vi "libssh2_agent_free.vi"(8 "error in (no error)":errorcluster, 11 "agent":T1) -> (0 "error out":errorcluster)   [LabVIEW 2017, in "libssh2.lvlib"]
doc: "Release memory associated with an SSH agent handle."
uses:
  libssh2.lvlib
  Agent Refnum.ctl
  Global Settings.vi
  Read Session Refnum.vi
  <vilib>/Utility/semaphor.llb/Acquire Semaphore.vi
  <vilib>/Utility/semaphor.llb/Release Semaphore.vi
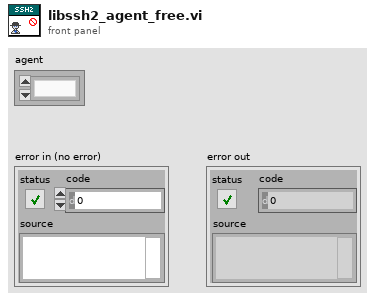
[diagram p1: front panel]
types:
  T1 = typedef "libssh2.lvlib/Agent Refnum.ctl" = refnum<k1>
  T2 = typedef "libssh2.lvlib/Session Refnum.ctl" = refnum<k1>
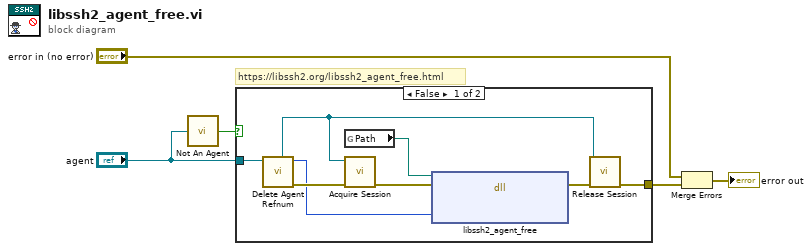
[diagram p0: block diagram]
diagram:
  # "https://libssh2.org/libssh2_agent_free.html"
  n1 = call "Not An Agent.vi"("agent"="agent") -> ("Not a Agent?"=w3:bool)
  n2 = case shown="False" w3 {
    tunnel: [w7 _] -> w5
    tunnel: "agent" -> [w9 _]
    frame False {
      n3 = call "Delete Agent Refnum.vi"("agent"=w9) -> ("error out"=w11:errorcluster, "LIBSSH2_AGENT*"=w10:u64, "session"=w6:T2)  [unwired: 8 in]
      n4 = global read "Global Settings.vi" "Path"() -> (w12:path)
      n5 = call "Acquire Session.vi"("error in (no error)"=w11, "session"=w6) -> ("error out"=w8:errorcluster)  [unwired: 7 in, 2 out]
      n6 = dll-call lib="?" fn="libssh2_agent_free"(path in=w12, error in=w8, "agent"=w10) -> (error out=w13:errorcluster)  [unwired: 3 in, 1 out]
      n7 = call "Release Session.vi"("error in (no error)"=w13, "session"=w6) -> ("error out"=w7:errorcluster)  [unwired: 9 in]
    }
    frame True {
    }
  }
  n8 = Merge Errors("error in (no error)", w5) -> (→"error out":errorcluster)
